vi "PuT3 DAQ.vi"(8 "error in":errorcluster, 10 "Ausgabewerte":dbl[](array[numeric]), 11 "Auftrag":T1={"Messart"=enum."Wahl treffen", "Kanal"="", "PFI"="", "Rate"=1000.0, "Samples"=100, "Bereich"=10.0, "Kontinuierlich"=FALSE}) -> (0 "error out":errorcluster, 1 "Status":dbl, 2 "Signal":waveform(dbl)(graph), 3 "Daten":dbl[](array[numeric]))   [LabVIEW 2026]
doc: "Virtuelles myDAQ. Auftrag und Ausgabewerte bedrahten. Daten sind Volt, Ohm, Hz oder Portwert je nach Messart. Signal ist eine analoge LabVIEW-Wellenform. Statuscodes stehen in der Anleitung."
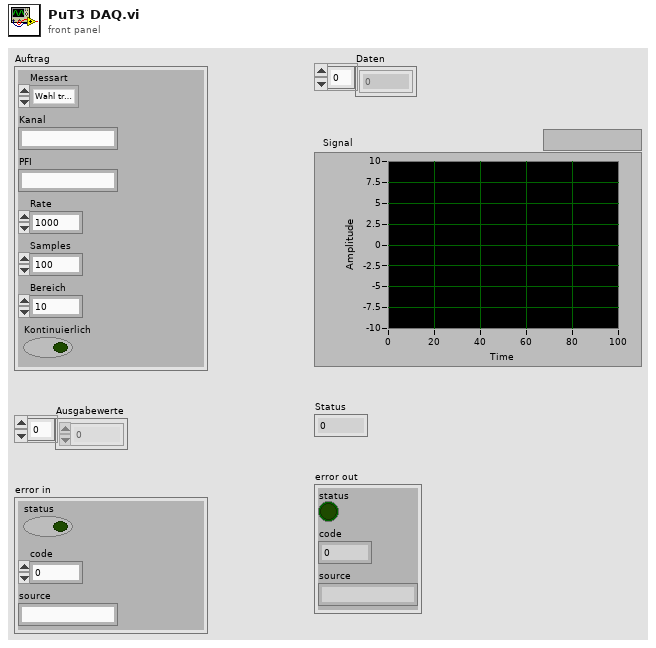
[diagram p1: front panel]
types:
  T1 = cluster{"Messart":enum8{"Wahl treffen", "AI Spannung", "AO Spannung", "DI Lesen", "DO Schreiben", "CTR Frequenz", "DMM Widerstand", "Ausgaenge freigeben"}, "Kanal":string, "PFI":string, "Rate":dbl, "Samples":i32, "Bereich":dbl, "Kontinuierlich":bool}
  T2 = enum8{"Wahl treffen", "AI Spannung", "AO Spannung", "DI Lesen", "DO Schreiben", "CTR Frequenz", "DMM Widerstand", "Ausgaenge freigeben"}
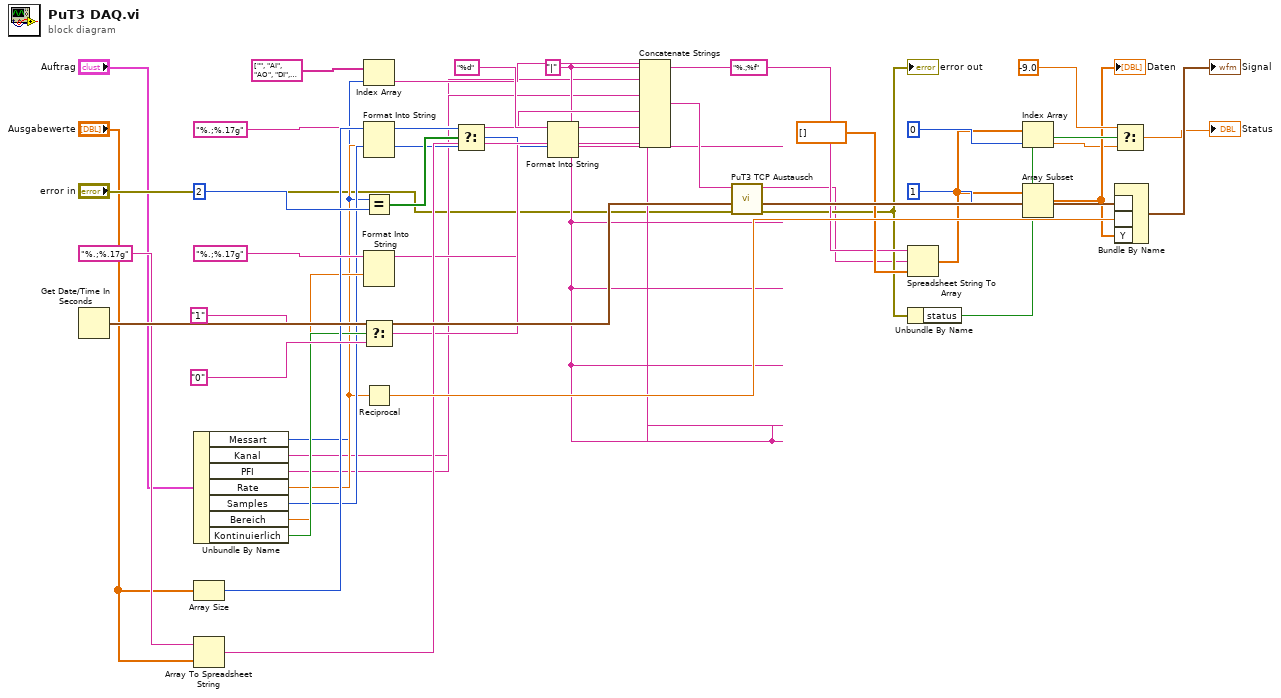
[diagram p0: block diagram]
diagram:
  w13 = "|"
  n1 = Get Date/Time In Seconds() -> (seconds since 1Jan1904=w43:timestamp)
  n2 = Unbundle By Name("Auftrag") -> ("Messart"=w4:T2, "Kanal"=w5:string, "PFI"=w6:string, "Rate"=w7:dbl, "Samples"=w8:i32, "Bereich"=w9:dbl, "Kontinuierlich"=w10:bool)
  n3 = Array Size(array="Ausgabewerte") -> (size(s)=w16:i32)
  n4 = Array To Spreadsheet String(array="Ausgabewerte", 3:"%.;%.17g") -> (spreadsheet string=w28:string)  [unwired: 1 in]
  n5 = Index Array(array=string[] ["", "AI", "AO", "DI", "DO", "FREQ", "OHM", "RESET"], index=w4) -> (element=w12:string)
  n6 = Format Into String(format string="%.;%.17g", w7) -> (resulting string=w15:string)  [unwired: 2 in, 1 out]
  n7 = Equal?(x=w4, y=u8 2) -> (x = y?=w18:bool[])
  n8 = Format Into String(format string="%.;%.17g", w9) -> (resulting string=w23:string)  [unwired: 2 in, 1 out]
  n9 = Select(t="1", s=w10, f="0") -> (s? t:f=w26:string)
  n10 = Reciprocal(x=w7) -> (1/x=w42:dbl)
  n11 = Select(t=w16, s=w18, f=w8) -> (s? t:f=w19:i32)
  n12 = Format Into String(format string="%d", w19) -> (resulting string=w21:string)  [unwired: 2 in, 1 out]
  n13 = Concatenate Strings(w12, w13, w5, w13, w6, w13, w15, w13, w21, w13, w23, w13, w26, w13, w28) -> (w29:string)
  n14 = call "PuT3 TCP Austausch.vi"("error in"="error in", "Anfrage"=w29) -> ("error out"=w31:errorcluster, "Antwort"=w30:string)  [unwired: 8 in]
  "error out" <- w31
  n15 = Spreadsheet String To Array(format string="%.;%f", spreadsheet string=w30, array type (2D Dbl)=dbl[] []) -> (array=w34:dbl[])  [unwired: 1 in]
  n16 = Unbundle By Name(w31) -> ("status"=w39:bool)
  n17 = Index Array(array=w34, index=0) -> (element=w36:dbl)
  n18 = Array Subset(array=w34, index=1) -> (w38:dbl[])  [unwired: 1 in]
  "Daten" <- w38
  n19 = Select(t=-9.0, s=w39, f=w36) -> (s? t:f=→"Status":dbl)
  n20 = Bundle By Name(w43, w42, "Y"=w38) -> (→"Signal":waveform(dbl))  [unwired: 1 in]
